vi "R_connection reference.vi"(8 "error in (no error)":errorcluster caption="错误输入（无错误）", 11 "Database_access输入":refnum<class "Database_access.lvclass">) -> (0 "error out":errorcluster caption="错误输出", 2 "connection reference":refnum<k1>, 3 "Database_access输出":refnum<class "Database_access.lvclass">)   [LabVIEW 2025, in "Database_access.lvclass"]
uses:
  Database_access.lvclass
  Database_access.lvclass/Database_access.ctl
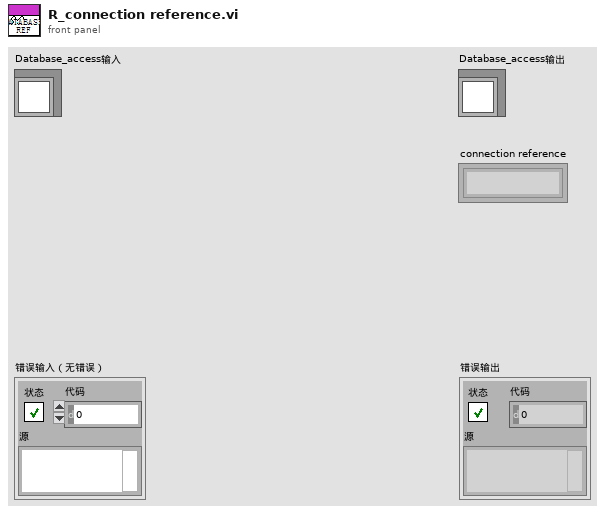
[diagram p1: front panel]
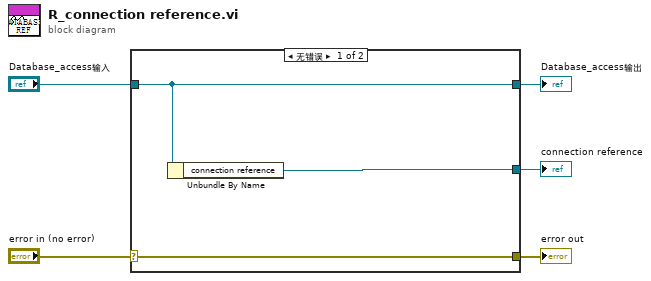
[diagram p0: block diagram]
diagram:
  n1 = case shown="无错误" "error in (no error)" {
    selector: "error in (no error)" -> [w8 w9]
    tunnel: [w8 w9] -> w4
    tunnel: [w7 w10] -> w2
    tunnel: "Database_access输入" -> [w7 w10]
    tunnel: [w6 _] -> w1
    frame No Error {
      n2 = Unbundle By Name(w7) -> ("connection reference"=w6:refnum<k1>)
    }
    frame Error {
    }
  }
  "error out" <- w4
  "Database_access输出" <- w2
  "connection reference" <- w1
